vi "mupDefineVar.vi"(8 "error in (no error)":errorcluster, 9 "initValue":dbl, 10 "varName":string, 11 "hParser in":u64) -> (0 "error out":errorcluster, 2 "varAddr":u64, 3 "hParser out":u64)   [LabVIEW 2018, in "mupLib.lvlib"]
doc: "Define a variable and set its initial value.\nThe variable's pointer is returned in varAddr."
uses:
  mupLib.lvlib
  <vilib>/Utility/error.llb/Error Cluster From Error Code.vi
  libmuparser-lv.dll
panel:
  # "Define a variable and set its initial value.\nThe variable's pointer is returned in varAddr."
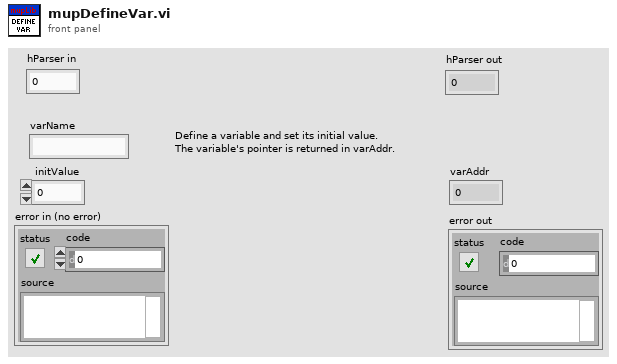
[diagram p1: front panel]
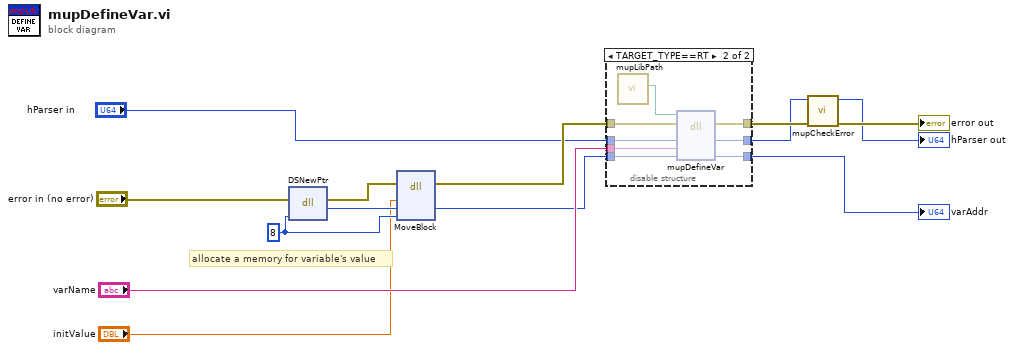
[diagram p0: block diagram]
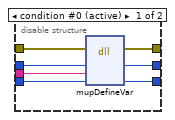
[diagram p2: hidden frame]
diagram:
  w13 = 8 ("size")
  # "allocate a memory for variable's value"
  n1 = dll-call lib="LabVIEW" fn="DSNewPtr"(error in="error in (no error)", "size"=w13) -> (error out=w12:errorcluster, "return type"=w14:u64)  [unwired: 3 in, 1 out]
  n2 = dll-call lib="LabVIEW" fn="MoveBlock"(error in=w12, "ps"="initValue", "pd"=w14, "size"=w13) -> (error out=w11:errorcluster, "pd"=w9:u64)  [unwired: 5 in, 1 out]
  n3 = disable-structure shown="TARGET_TYPE==RT" {
    disable-tunnel: w11 -> [w21 w29]
    disable-tunnel: "varName" -> [w20 w28]
    disable-tunnel: w9 -> [w19 w27]
    disable-tunnel: [w18 w26] -> w8
    disable-tunnel: [w17 w25] -> w6
    disable-tunnel: "hParser in" -> [w16 w24]
    disable-tunnel: [w15 w23] -> w2
    frame condition #0 (active) {
      n4 = dll-call lib="C:/Users/leonidas/Documents/GitHub/LV-muParser/mupLib/libmuparser-lv.dll" fn="mupDefineVar"(error in=w21, "hParser"=w16, "szName"=w20, "fVar"=w19) -> (error out=w17:errorcluster, "hParser"=w15:u64, "fVar"=w18:u64)  [unwired: 4 in, 1 out]
    }
    frame condition #1 {
      n5 = call "mupLibPath.vi"() -> ("libmuparser path"=w22:path)  [unwired: 11 in]
      n6 = dll-call lib="C:/Users/leonidas/Documents/GitHub/LV-muParser/mupLib/libmuparser-lv.dll" fn="mupDefineVar"(path in=w22, error in=w29, "hParser"=w24, "szName"=w28, "fVar"=w27) -> (error out=w25:errorcluster, "hParser"=w23:u64, "fVar"=w26:u64)  [unwired: 3 in, 1 out]
    }
  }
  "varAddr" <- w8
  n7 = call "mupCheckError.vi"("error in (no error)"=w6, "hParser in"=w2) -> ("error out"=→"error out":errorcluster, "hParser out"=→"hParser out":u64)  [unwired: 8 in]
